vi "set Channel Measurement Bandwidth.vi"(6 "Target Channel Type":T1(ring) caption="Channel (TX Channel)", 8 "error in (no error)":errorcluster, 9 "TX Channel Index":i32=1 min=1, 10 "Channel BandWidth (Hz)":dbl, 11 "FSV-40N in":refnum<class "FSV-40N.lvclass">) -> (0 "error out":errorcluster, 3 "FSV-40N out":refnum<class "FSV-40N.lvclass">)   [LabVIEW 2023, in "Spectrum Analyzer.lvlib" / "FSV-40N.lvclass"]
uses:
  FSV-40N.lvclass
  FSV-40N.lvclass/FSV-40N.ctl
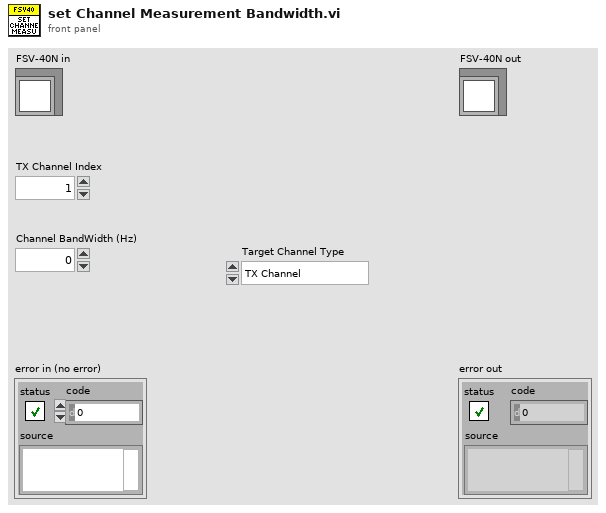
[diagram p1: front panel]
types:
  T1 = enum16{"TX Channel", "Adjacent Channel", "Alternate Channel"}
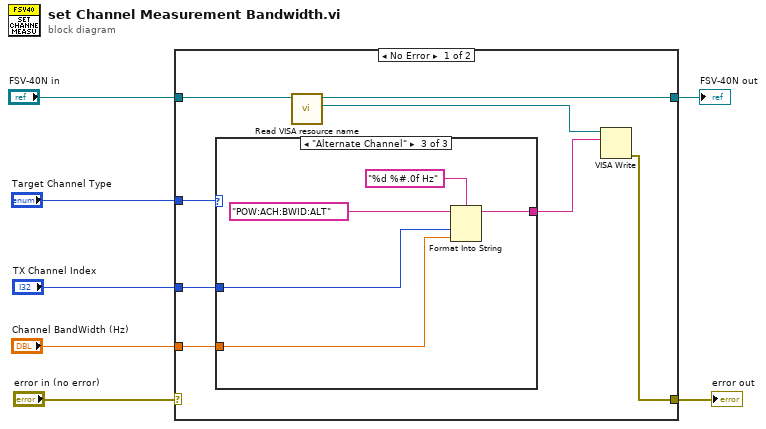
[diagram p0: block diagram]
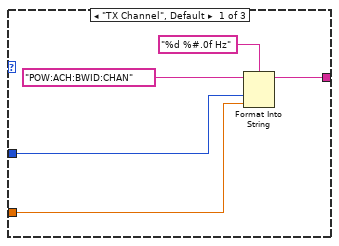
[diagram p2: hidden frame]
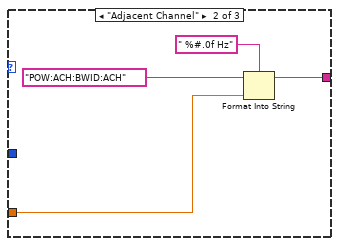
[diagram p3: hidden frame]
diagram:
  n1 = case shown="No Error" "error in (no error)" {
    selector: "error in (no error)" -> [_ w30]
    tunnel: "FSV-40N in" -> [w15 w31]
    tunnel: [w13 w31] -> w6
    tunnel: [w12 w30] -> w4
    tunnel: "TX Channel Index" -> [w10 _]
    tunnel: "Channel BandWidth (Hz)" -> [w9 _]
    tunnel: "Target Channel Type" -> [w8 _]
    frame No Error {
      n2 = case shown="\"Alternate Channel\"" w8 {
        tunnel: [w18 w22 w27] -> w11
        tunnel: w10 -> [w17 _ w26]
        tunnel: w9 -> [w16 w21 w25]
        frame "TX Channel", Default {
          n3 = Format Into String(format string="%d %#.0f Hz", initial string="POW:ACH:BWID:CHAN", w17, w16) -> (resulting string=w18:string)  [unwired: 1 in, 1 out]
        }
        frame "Adjacent Channel" {
          n4 = Format Into String(format string=" %#.0f Hz", initial string="POW:ACH:BWID:ACH", w21) -> (resulting string=w22:string)  [unwired: 1 in, 1 out]
        }
        frame "Alternate Channel" {
          n5 = Format Into String(format string="%d %#.0f Hz", initial string="POW:ACH:BWID:ALT", w26, w25) -> (resulting string=w27:string)  [unwired: 1 in, 1 out]
        }
      }
      n6 = call "Read VISA resource name.vi"("FSV-40N in"=w15) -> ("VISA resource name"=w14:refnum<visa-resource-name>, "FSV-40N out"=w13:refnum<class "FSV-40N.lvclass">)  [unwired: 8 in, 1 out]
      n7 = VISA Write(VISA resource name=w14, write buffer=w11) -> (error out=w12:errorcluster)  [unwired: 1 in, 2 out]
    }
    frame Error {
    }
  }
  "error out" <- w4
  "FSV-40N out" <- w6
